vi "VM3 - DBL Scalar.vi"(5 "cmd (read)":enum16{"create", "destroy", "write", "read"}(ring)=enum."read", 7 "VC Handle":T2, 8 "error in":errorcluster, 9 "writer ID":u32, 10 "value in":dbl, 11 "name_spec":string) -> (0 "error out":errorcluster, 1 "stats":T1, 2 "value out":dbl, 3 "dup name_spec":string)   [LabVIEW 2021]
doc: "This VI manages variables of the <b>DBL Number</b> data type. Refer to the VI Help for more details.\n\n<b>cmd (read)</b> specifies the operation to perform on the variable: create, write, read, or destroy.\n\n<b>VC Handle</b> specifies the handle of the variable context. To operate on a global variable, pass -1 to this input. <b>name_spec</b> is the name specifier of the desired variable; usually, it is merely a variable name (see the VI Help for more options).\n\n<b>value in</b> and <b>value out</b> are the input and output values written to or read from the variable, respectively.\n\n<b>writer ID</b> specifies the Writer ID to be set along with the new value when writing or creating a variable.\n\n<b>stats</b> returns information about the most recent value of the variable, such as its Writer ID, update time, and update counter.\n\n::: CalcExpress Toolkit :::\nCopyright (c) 2000-2026 Konstantin Shifershteyn. All rights reserved."
uses:
  cetypes.llb/VarMan Variable Context Handle.ctl
  cetypes.llb/VarMan Variable Data Statistics.ctl
  cetypes.llb/VarMan Error Code.ctl
  cersrc/celveng32.dll
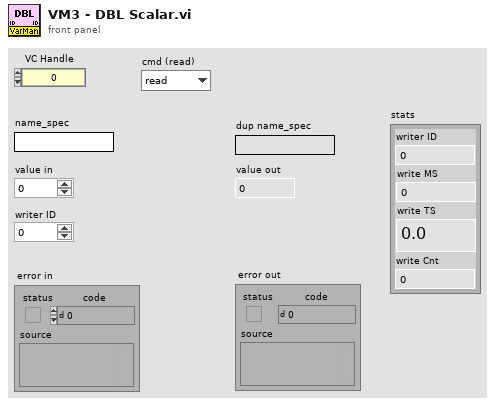
[diagram p1: front panel]
types:
  T1 = typedef "VarMan Variable Data Statistics.ctl" = cluster{"writer ID":u32, "write MS":u32, "write TS":dbl, "write Cnt":u32}
  T2 = typedef "VarMan Variable Context Handle.ctl" = i32
  T3 = typedef "VarMan Error Code.ctl" = u16
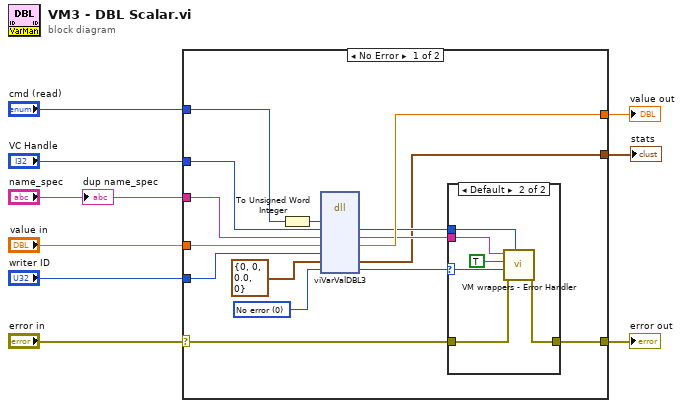
[diagram p0: block diagram]
diagram:
  n1 = case shown="No Error" "error in" {
    selector: "error in" -> [w19 w33]
    tunnel: [w24 w32] -> w4
    tunnel: "value in" -> [w23 w32]
    tunnel: "cmd (read)" -> [w22 _]
    tunnel: "name_spec" -> [w21 _]
    tunnel: "VC Handle" -> [w15 _]
    tunnel: [w20 w33] -> w5
    tunnel: "writer ID" -> [w14 _]
    tunnel: [w10 _] -> w1
    frame No Error {
      w16 = T3 0 items=["No error", "Invalid variable type", "Variable not found", "Variable already exists", "Invalid context handle", "Input error", "Invalid data format", "No history attached", "History already attached", "Invalid history parameters", "Wrong variable name", "Wrong alias name", "Non-unique alias", "Alias not found", "No alias associated", "Alias already associated", "Wrong context name", "Non-unique context name", "Context name not found", "Invalid parameter", "Generic error", "Memory Full", "Unrecognized LV error", "Unknown error code"] ("err code")
      n2 = To Unsigned Word Integer(number=w22) -> (unsigned 16bit integer=w18:u16)
      n3 = dll-call lib="C:/LV Projects/CalcExpress 40 LV2021/vi.lib/addons/CalcExpress/cersrc/celveng*.dll" fn="viVarValDBL3"("cmd"=w18, "vch"=w15, "name"=w21, "value"=w23, "writerID"=w14, "wrStats"=T1 {"writer ID"=0, "write MS"=0, "write TS"=0.0, "write Cnt"=0} ("stats"), "errc"=w16) -> ("vch"=w12:i32, "name"=w13:string, "value"=w24:dbl, "wrStats"=w10:T1, "errc"=w17:T3)  [unwired: 6 in, 2 out]
      n4 = case shown="Default" w17 {
        selector: w17 -> [_ w28]
        tunnel: [w25 w31] -> w20
        tunnel: w19 -> [w25 w30]
        tunnel: w13 -> [_ w27]
        tunnel: w12 -> [_ w26]
        frame 0 {
        }
        frame Default {
          n5 = call "VM wrappers - Error Handler.vi"("VC Handle"=w26, "error before"=w30, "VarMan error"=w28, "show name spec (F)"=TRUE, "name spec"=w27) -> ("error out"=w31:errorcluster)  [unwired: 5 in, 1 out]
        }
      }
    }
    frame Error {
    }
  }
  "value out" <- w4
  "error out" <- w5
  "stats" <- w1
  "dup name_spec" <- "name_spec"
